vi "JobDetailMap.Add KeyValue.vi"(8 "error in (no error)":errorcluster, 9 "Value":variant, 10 "Key":string, 11 "Job in":refnum<class "Job.lvclass">) -> (0 "error out":errorcluster, 3 "Job out":refnum<class "Job.lvclass">)   [LabVIEW 2013, in "openCronJob.lvlib" / "Job.lvclass"]
uses:
  Job.lvclass
  Job.lvclass/Job.ctl
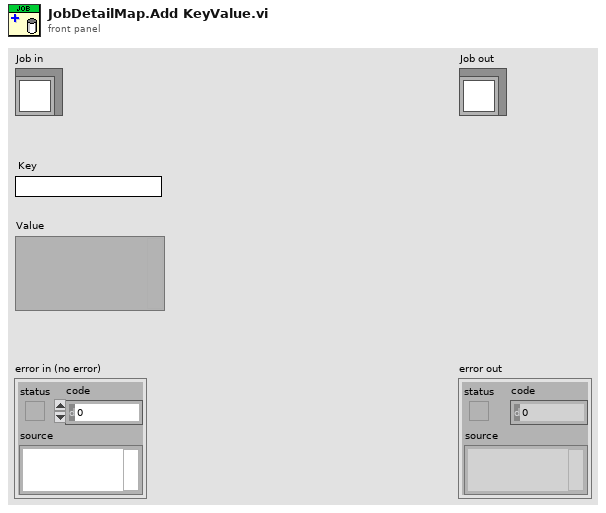
[diagram p1: front panel]
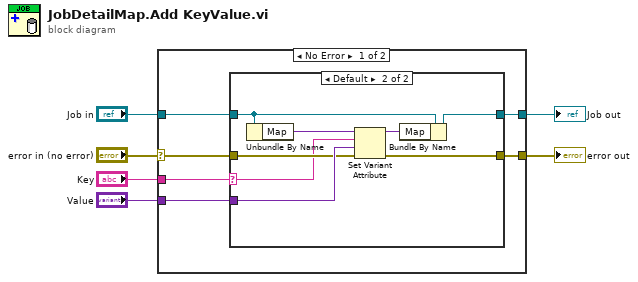
[diagram p0: block diagram]
diagram:
  n1 = case shown="No Error" "error in (no error)" {
    selector: "error in (no error)" -> [w11 w24]
    tunnel: [w10 w24] -> w5
    tunnel: [w9 w23] -> w3
    tunnel: "Job in" -> [w8 w23]
    tunnel: "Key" -> [w7 _]
    tunnel: "Value" -> [w12 _]
    frame No Error {
      n2 = case shown="Default" w7 {
        selector: w7 -> [_ w15]
        tunnel: w12 -> [_ w21]
        tunnel: w11 -> [w13 w19]
        tunnel: [w13 w18] -> w10
        tunnel: [w14 w17] -> w9
        tunnel: w8 -> [w14 w16]
        frame "" {
        }
        frame Default {
          n3 = Unbundle By Name(w16) -> ("Map"=w22:variant)
          n4 = Set Variant Attribute(Variant=w22, name=w15, value=w21, error in=w19) -> (Variant out=w20:variant, error out=w18:errorcluster)  [unwired: 1 out]
          n5 = Bundle By Name(cluster=w16, "Map"=w20) -> (w17:refnum<class "Job.lvclass">)
        }
      }
    }
    frame Error {
    }
  }
  "error out" <- w5
  "Job out" <- w3
